vi "Test_C_Decode_To_Frames.vi"() -> ()   [LabVIEW 2021]
doc: "A2 test, no device: encodes n test frames (W10), decodes the stream in two pieces (cut at) with W13 C_Decode_RT and with C_Decode_To_Frames, and compares result, frames and decoder state after each piece (Compare Aggregates). pass = all equal."
uses:
  CANsub_C.lvlib
  C_RX_State.ctl
  api/Typedefs/CANsub_Frames.ctl
  api/CANsub_API.lvlib
panel:
  out "error out":errorcluster
  out "stream length":i32
  out "n frames per call":i32[](array[numeric])
  in  "cut at":i32=17
  in  "n test frames":i32=5
  out "pass":bool
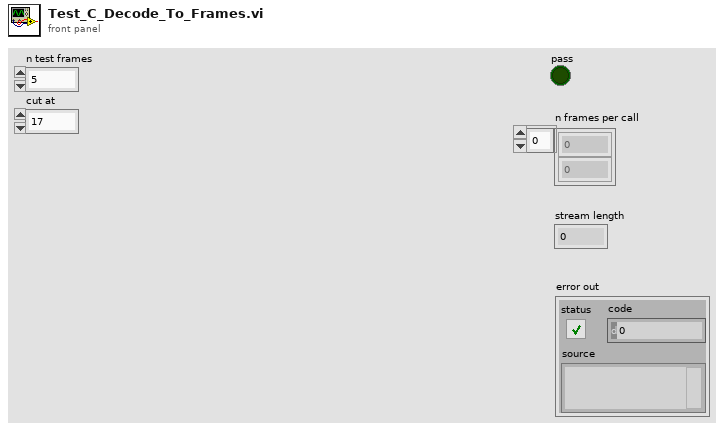
[diagram p1: front panel]
types:
  T1 = typedef "CANsub_API.lvlib/CANsub_Frames.ctl" = cluster{"count":i32, "t_dev":dbl[], "id":u32[], "flags":u16[], "dlc":u8[], "data len":u8[], "data":u8[]}
  T2 = typedef "CANsub_C.lvlib/C_RX_State.ctl" = cluster{"ws":u8[], "hdlc":u8[], "ping":u8[]}
  T3 = typedef "CANsub_C.lvlib/C_RX_Buffers.ctl" = cluster{"t_dev":dbl[], "ws":u8[], "id":u32[], "flags":u16[], "hdlc":u8[], "dlc":u8[], "data len":u8[], "data":u8[], "ping":u8[]}
  T4 = typedef "CANsub_C.lvlib/C_Decode_Result.ctl" = cluster{"n frames":i32, "peer close":bool, "ping len":i32, "crc errors":u32, "decode errors":i32}
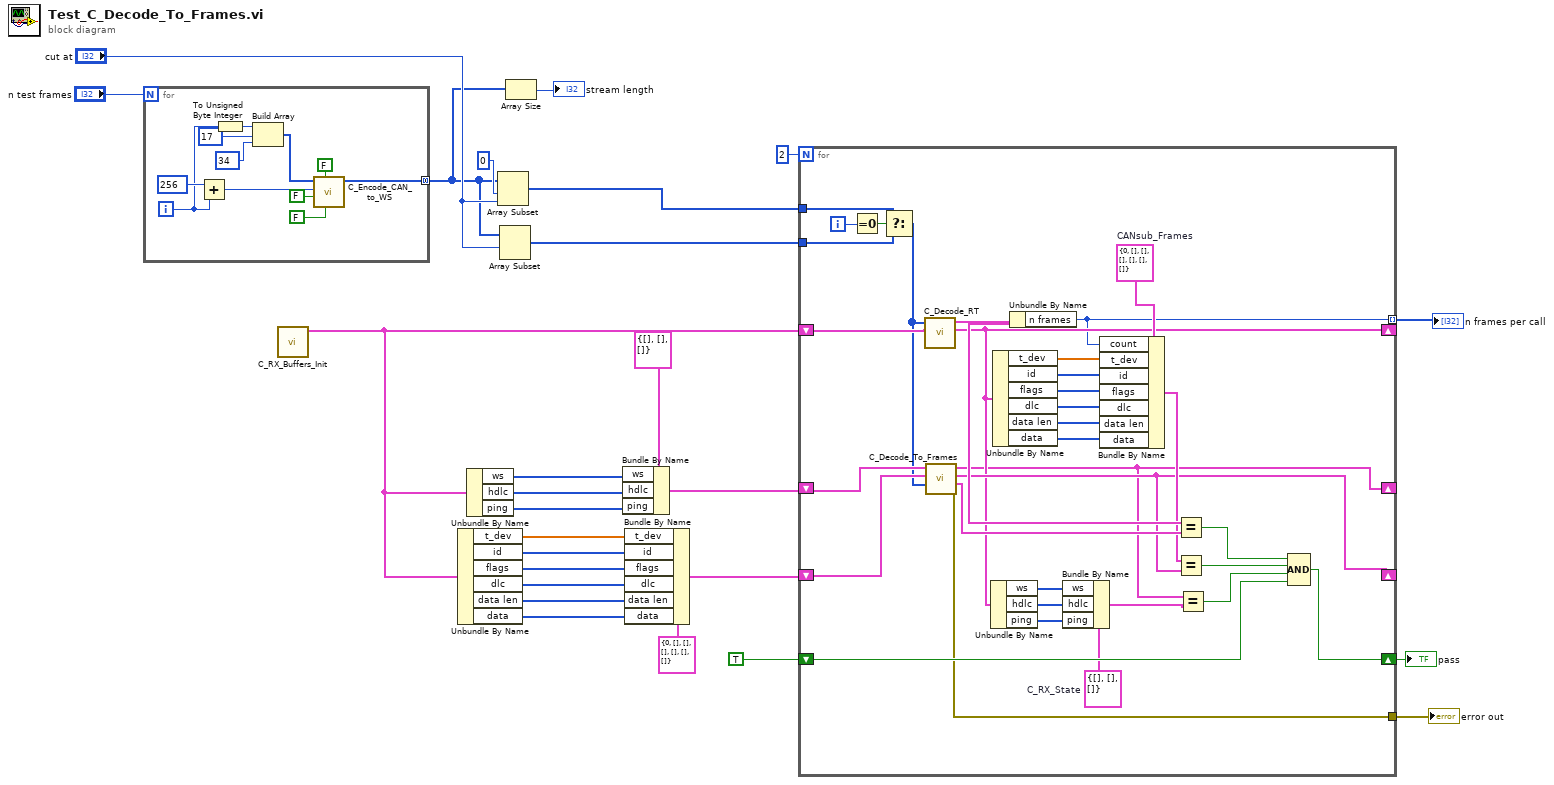
[diagram p0: block diagram]
diagram:
  n1 = for {
    N: "n test frames" -> [_]
    tunnel: [w27] -> w1 mode=concatenating
    i -> [w34]
    n2 = Add(x=u32 256, y=w34) -> (x+y=w36:u32)
    n3 = To Unsigned Byte Integer(number=w34) -> (unsigned 8bit integer=w35:u8)
    n4 = Build Array(w35, u8 17 ("element"), u8 34 ("element")) -> (w31:u8[])
    n5 = call "C_Encode_CAN_to_WS.vi"("brs"=FALSE, "ide"=FALSE, "fdf"=FALSE, "id"=w36, "data"=w31) -> ("ws frame"=w27:u8[])  [unwired: 5 in, 1 out]
  }
  n6 = call "C_RX_Buffers_Init.vi"() -> ("buffers"=w10:T3)  [unwired: 8 in, 3 out]
  n7 = Unbundle By Name(w10) -> ("t_dev"=w19:dbl[], "id"=w18:u32[], "flags"=w17:u16[], "dlc"=w16:u8[], "data len"=w15:u8[], "data"=w14:u8[])
  n8 = Unbundle By Name(w10) -> ("ws"=w23:u8[], "hdlc"=w22:u8[], "ping"=w21:u8[])
  n9 = Array Subset(array=w1, index=0, length="cut at") -> (w6:u8[])
  n10 = Array Subset(array=w1, index="cut at") -> (w5:u8[])  [unwired: 1 in]
  n11 = Array Size(array=w1) -> (size(s)=→"stream length":i32)
  n12 = Bundle By Name(cluster=T2 {"ws"=[], "hdlc"=[], "ping"=[]} ("C_RX_State"), "ws"=w23, "hdlc"=w22, "ping"=w21) -> (w12:T2)
  n13 = Bundle By Name(cluster=T1 {"count"=0, "t_dev"=[], "id"=[], "flags"=[], "dlc"=[], "data len"=[], "data"=[]} ("CANsub_Frames"), "t_dev"=w19, "id"=w18, "flags"=w17, "dlc"=w16, "data len"=w15, "data"=w14) -> (w11:T1)
  n14 = for {
    N: 2 -> [_]
    shift-right: [w40] -> _
    shift-left: w12 -> [w60]
    shift-right: [w47] -> _
    shift-left: w11 -> [w59]
    shift-right: [w46] -> _
    shift-left: w10 -> [w61]
    shift-right: [w66] -> w8
    shift-left: TRUE -> [w67]
    tunnel: w6 -> [w63]
    tunnel: w5 -> [w62]
    tunnel: [w39] -> w4
    tunnel: [w38] -> w3 mode=indexing
    i -> [w64]
    w45 = T2 {"ws"=[], "hdlc"=[], "ping"=[]}  # C_RX_State
    w56 = T1 {"count"=0, "t_dev"=[], "id"=[], "flags"=[], "dlc"=[], "data len"=[], "data"=[]}  # CANsub_Frames
    n15 = Equal To 0?(x=w64) -> (x = 0?=w65:bool)
    n16 = Select(t=w63, s=w65, f=w62) -> (s? t:f=w58:u8[])
    n17 = call "C_Decode_RT.vi"("buffers in"=w61, "bytes in"=w58) -> ("buffers out"=w46:T3, "result"=w55:T4)  [unwired: 7 in, 1 out]
    n18 = call "C_Decode_To_Frames.vi"("bytes in"=w58, "frames in"=w59, "state in"=w60) -> ("error out"=w39:errorcluster, "result"=w57:T4, "frames out"=w47:T1, "state out"=w40:T2)  [unwired: 5 in]
    n19 = Unbundle By Name(w46) -> ("ws"=w44:u8[], "hdlc"=w43:u8[], "ping"=w42:u8[])
    n20 = Unbundle By Name(w46) -> ("t_dev"=w54:dbl[], "id"=w53:u32[], "flags"=w52:u16[], "dlc"=w51:u8[], "data len"=w50:u8[], "data"=w49:u8[])
    n21 = Unbundle By Name(w55) -> ("n frames"=w38:i32)
    n22 = Bundle By Name(cluster=w45, "ws"=w44, "hdlc"=w43, "ping"=w42) -> (w41:T2)
    n23 = Bundle By Name(cluster=w56, "count"=w38, "t_dev"=w54, "id"=w53, "flags"=w52, "dlc"=w51, "data len"=w50, "data"=w49) -> (w48:T1)
    n24 = Equal?(x=w55, y=w57) -> (x = y?=w70:bool)
    n25 = Equal?(x=w48, y=w47) -> (x = y?=w69:bool)
    n26 = Equal?(x=w40, y=w41) -> (x = y?=w68:bool)
    n27 = Compound Arithmetic op=AND(w70, w69, w68, w67) -> (w66:bool)
  }
  "pass" <- w8
  "error out" <- w4
  "n frames per call" <- w3
